vi "NEO Set Pod Setpoints.vi"(8 "Steer Angles (degrees)":T3, 9 "Drive Velocities (ft/s)":T3, 10 "Pod Setpoints (ft/s and deg)":T8, 11 "Motors In":T4 {"Steer Scaling" format="%.2f"; "Drive Scaling" format="%.2f"; "Pod Locations (ft)"."Right Back" format="%.2f"; "Pod Locations (ft)"."Right Front" format="%.2f"; "Pod Locations (ft)"."Left Back" format="%.2f"; "Pod Locations (ft)"."Left Front" format="%.2f"}) -> (3 "Arbitrary":T2(graph))   [LabVIEW 2023]
uses:
  4b768f86-8279-4062-bf26-12cbbaf62c6c.vi
  <vilib>/REV Custom Controls/Spark Output Control Type.ctl
  <vilib>/REVLibDriver/REVLibDriver.lvlib
  Type Definitions/Data/Pod Setpoints.ctl
  Type Definitions/Data/Pod Positions.ctl
  Type Definitions/Hardware/Swerve Drives/(NEO-NEO-ThroughBore-Pigeon2) Swerve.ctl
  <vilib>/REV Custom Controls/REVSparkRefnum.ctl
panel:
  out "Setpoints Out":dbl[](array[numeric])
  in  "PID Gains":T1
  in  "Motor Type":enum16{"Drive", "Steer"}(ring)
  in  "Motor Position":T7(ring)
  out "PID Graph":cluster{"Left Front":dbl, "Theta":dbl}(graph)
  out "Values":cluster{"Actual":dbl, "Setpoint":dbl}
  in  "Debug Mode?":bool
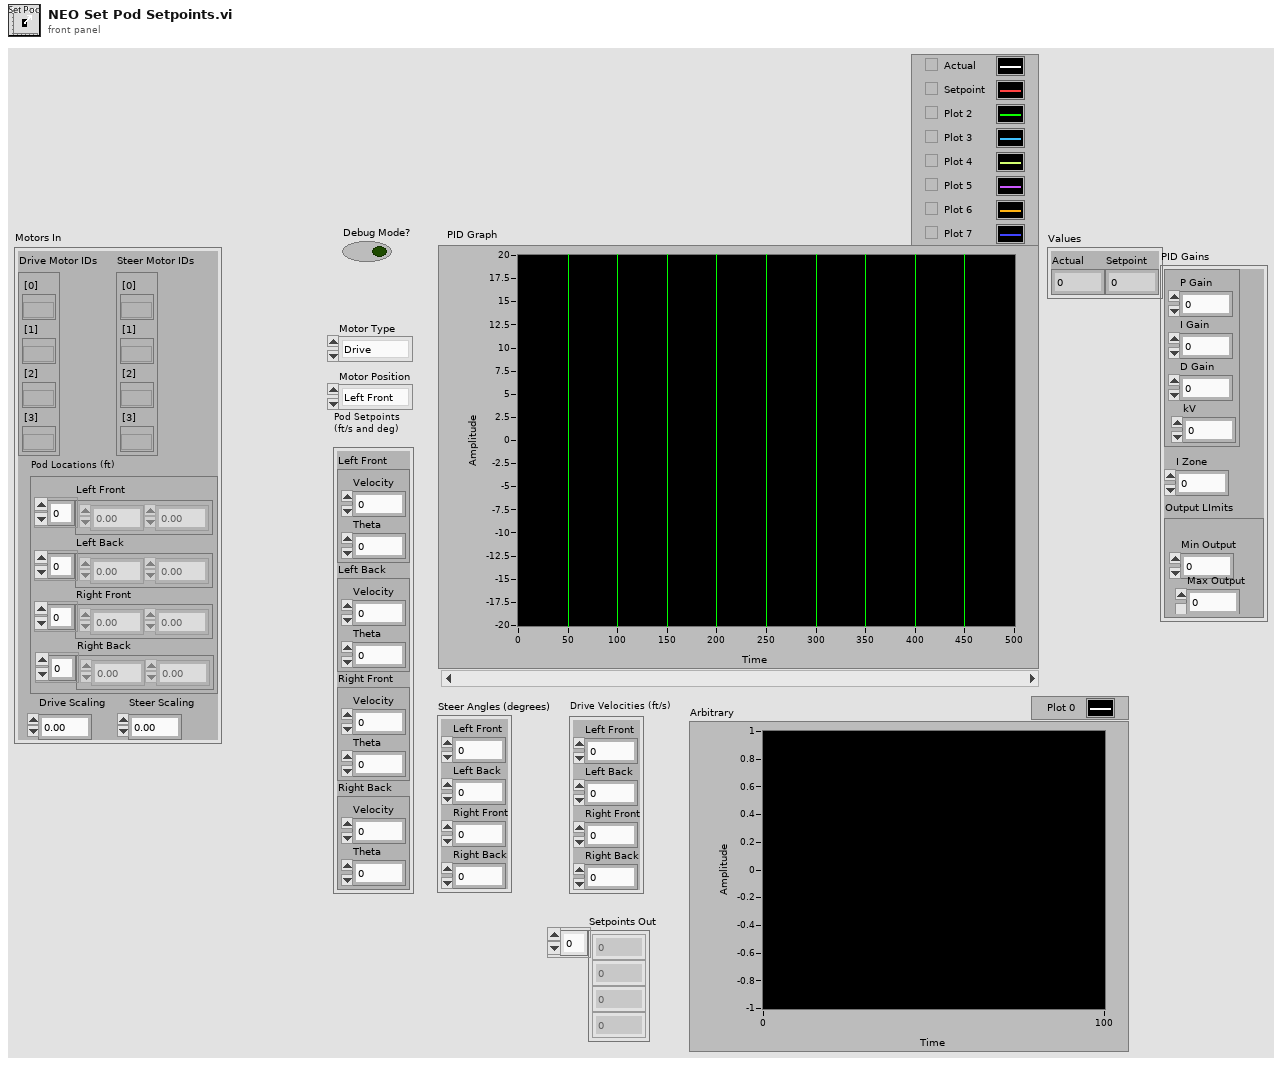
[diagram p1: front panel]
types:
  T1 = cluster{cluster{"P Gain":dbl, "I Gain":dbl, "D Gain":dbl, "kV":dbl}, "I Zone":dbl, "Output LImits":cluster{"Min Output":dbl, "Max Output":dbl}}
  T2 = cluster{"[0]":dbl, "[1]":dbl, "[2]":dbl, "[3]":dbl}
  T3 = cluster{"Left Front":dbl, "Left Back":dbl, "Right Front":dbl, "Right Back":dbl}
  T4 = typedef "(NEO-NEO-ThroughBore-Pigeon2) Swerve.ctl" = cluster{"Drive Motor IDs":cluster{"[0]":T5, "[1]":T5, "[2]":T5, "[3]":T5}, "Steer Motor IDs":cluster{"[0]":T5, "[1]":T5, "[2]":T5, "[3]":T5}, "Pod Locations (ft)":T6, "Drive Scaling":dbl, "Steer Scaling":dbl}
  T5 = typedef "REVLibDriver.lvlib/REVSparkRefnum.ctl" = refnum<k20>
  T6 = typedef "Pod Positions.ctl" = cluster{"Left Front":dbl[], "Left Back":dbl[], "Right Front":dbl[], "Right Back":dbl[]}
  T7 = enum16{"Left Front", "Left Back", "Right Front", "Right Back"}
  T8 = typedef "Pod Setpoints.ctl" = cluster{"Left Front":cluster{"Velocity":dbl, "Theta":dbl}, "Left Back":cluster{"Velocity":dbl, "Theta":dbl}, "Right Front":cluster{"Velocity":dbl, "Theta":dbl}, "Right Back":cluster{"Velocity":dbl, "Theta":dbl}}
  T9 = typedef "REVLibDriver.lvlib/Spark Output Control Type.ctl" = enum16{"Percent VBus", "Velocity", "Voltage", "Position", "Current", "MAXMotion Position", "MAXMotion Velocity"}
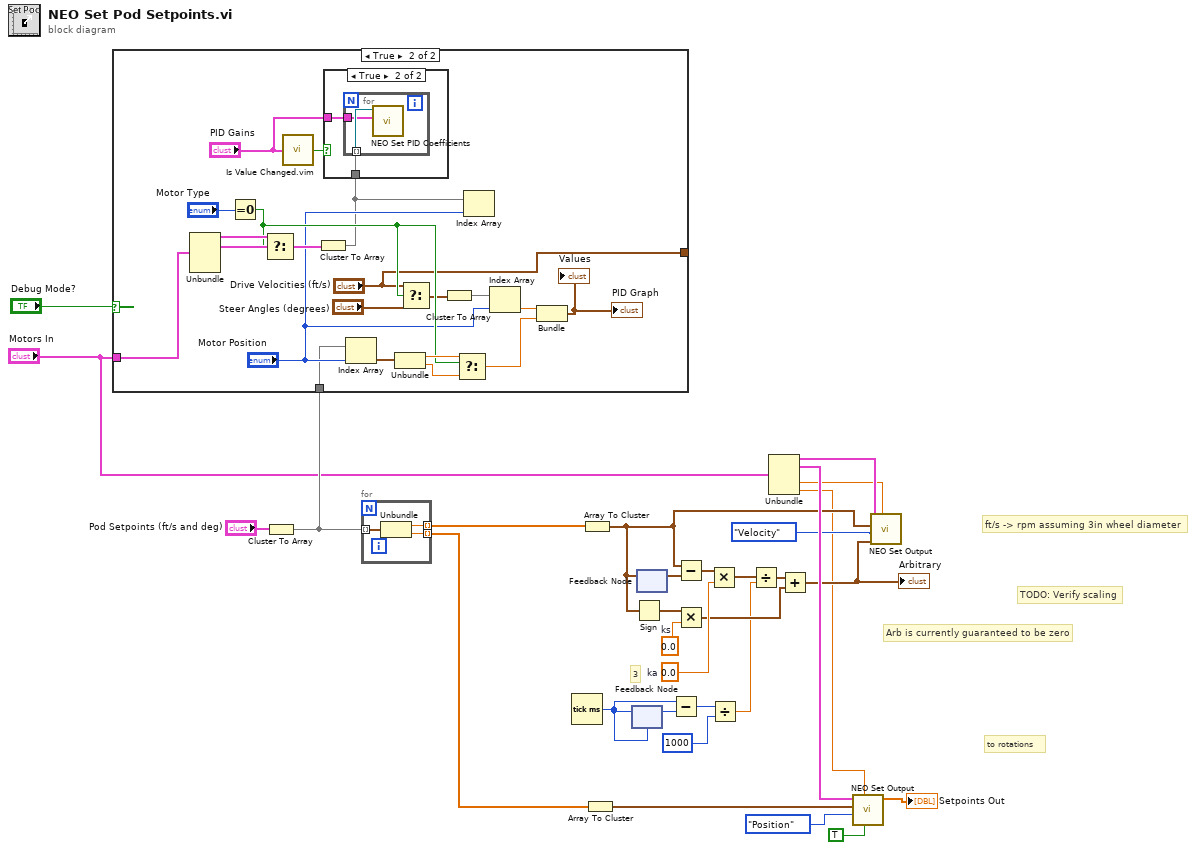
[diagram p0: block diagram]
diagram:
  w25 = 0.0  # ka
  w23 = 0.0  # ks
  # "Arb is currently guaranteed to be zero"
  # "to rotations"
  # "ft/s -> rpm assuming 3in wheel diameter"
  # "TODO: Verify scaling"
  # "3"
  n1 = Cluster To Array(cluster="Pod Setpoints (ft/s and deg)") -> (array=w28:cluster{"Velocity":dbl, "Theta":dbl}[])
  n2 = case shown="True" "Debug Mode?" {
    tunnel: "Motors In" -> [_ w42]
    tunnel: w28 -> [_ w33]
    tunnel: [_ "Drive Velocities (ft/s)"] -> _
    frame False {
    }
    frame True {
      n3 = Unbundle(w42) -> ("Drive Motor IDs"=w50:cluster{"[0]":T5, "[1]":T5, "[2]":T5, "[3]":T5}, "Steer Motor IDs"=w49:cluster{"[0]":T5, "[1]":T5, "[2]":T5, "[3]":T5})  [unwired: 3 out]
      n4 = Equal To 0?(x="Motor Type") -> (x = 0?=w46:bool)
      n5 = Select(t=w50, s=w46, f=w49) -> (s? t:f=w41:cluster{"[0]":T5, "[1]":T5, "[2]":T5, "[3]":T5})
      n6 = call "Is Value Changed.vim"("value"="PID Gains") -> ("changed or first call?"=w37:bool)
      n7 = Cluster To Array(cluster=w41) -> (array=w36:T5[])
      n8 = case shown="True" w37 {
        tunnel: w36 -> [_ w53]
        tunnel: "PID Gains" -> [_ w52]
        frame False {
        }
        frame True {
          n9 = for {
            tunnel: w53 -> [w55] mode=indexing
            tunnel: w52 -> [w54]
            n10 = call "NEO Set PID Coefficients.vi"("PID Gains"=w54, "Spark refnum"=w55) -> ()  [unwired: 6 in, 2 out]
          }
        }
      }
      n11 = Index Array(array=w33, index="Motor Position") -> (element=w34:cluster{"Velocity":dbl, "Theta":dbl})
      n12 = Unbundle(w34) -> ("Velocity"=w48:dbl, "Theta"=w47:dbl)
      n13 = Select(t="Drive Velocities (ft/s)", s=w46, f="Steer Angles (degrees)") -> (s? t:f=w45:T3)
      n14 = Cluster To Array(cluster=w45) -> (array=w32:dbl[])
      n15 = Select(t=w48, s=w46, f=w47) -> (s? t:f=w43:dbl)
      n16 = Index Array(array=w36, index="Motor Position") -> ()  [unwired: 1 out]
      n17 = Index Array(array=w32, index="Motor Position") -> (element=w44:dbl)
      n18 = Bundle("Left Front"=w44, "Theta"=w43) -> (→"PID Graph" →"Values":cluster{"Left Front":dbl, "Theta":dbl})  [unwired: 1 in]
    }
  }
  n19 = for {
    tunnel: w28 -> [w58] mode=indexing
    tunnel: [w57] -> w3 mode=indexing
    tunnel: [w56] -> w2 mode=indexing
    n20 = Unbundle(w58) -> ("Velocity"=w57:dbl, "Theta"=w56:dbl)
  }
  n21 = Tick Count (ms)() -> (millisecond timer value=w12:u32)
  n22 = Array To Cluster(array=w3) -> (cluster=w17:T2)
  n23 = Array To Cluster(array=w2) -> (cluster=w18:T2)
  n24 = feedback #1(w12) -> (w11:u32)
  n25 = feedback-in #1(w12) -> ()
  n26 = Sign(1:w17) -> (0:w24:T2)
  n27 = feedback #2() -> (w26:T2)  [unwired: 1 in]
  n28 = feedback-in #2(w17) -> ()
  n29 = Subtract(x=w12, y=w11) -> (x-y=w13:u32)
  n30 = Subtract(x=w17, y=w26) -> (x-y=w20:T2)
  n31 = Multiply(x=w24, y=w23) -> (x*y=w22:T2)
  n32 = Multiply(x=w20, y=w25) -> (x*y=w9:T2)
  n33 = Divide(x=w13, y=u32 1000) -> (x/y=w8:dbl)
  n34 = Divide(x=w9, y=w8) -> (x/y=w10:T2)
  n35 = Unbundle("Motors In") -> ("Drive Motor IDs"=w27:cluster{"[0]":T5, "[1]":T5, "[2]":T5, "[3]":T5}, "Steer Motor IDs"=w21:cluster{"[0]":T5, "[1]":T5, "[2]":T5, "[3]":T5}, "Drive Scaling"=w5:dbl, "Steer Scaling"=w4:dbl)  [unwired: 1 out]
  n36 = Add(x=w10, y=w22) -> (x+y=w15:T2)
  "Arbitrary" <- w15
  n37 = call "NEO Set Output.vi"("Add Angle Offsets?"=TRUE, "Scaling"=w4, "Control Mode"=Spark_Output_Control_Type."Position", "Setpoints"=w18, "Motors"=w21) -> ("Setpoints Out"=→"Setpoints Out":dbl[])  [unwired: 6 in]
  n38 = call "NEO Set Output.vi"("Scaling"=w5, "Arbitrary Feedforward"=w15, "Control Mode"=Spark_Output_Control_Type."Velocity", "Setpoints"=w17, "Motors"=w27) -> ()  [unwired: 6 in, 1 out]
